vi "Write CE BT Hop Number Setting.vi"(8 "error in (no error)":errorcluster, 10 "CE BT Hop Number Setting":T1 {"Start/Stop Frequency(Hz)"."Stop" format="%#_6p"; "Start/Stop Frequency(Hz)"."Start" format="%#_6p"; "Sweep Time(s)"."Time" format="%#_6p"; "RBW/VBW(Hz)"."VBW" format="%#_6p"; "RBW/VBW(Hz)"."RBW" format="%#_6p"}, 11 "SA Measurement in":refnum<class "SA Measurement.lvclass">) -> (0 "error out":errorcluster, 3 "SA Measurement out":refnum<class "SA Measurement.lvclass">)   [LabVIEW 2023, in "Spectrum Analyzer.lvlib" / "SA Measurement.lvclass"]
uses:
  SA Measurement.lvclass
  SA Measurement.lvclass/SA Measurement.ctl
  TYPE DEFINITION/TYPE Reference Level and Atten Param.ctl
  Spectrum Analyzer.lvlib
  TYPE DEFINITION/TYPE Y-axis Unit.ctl
  TYPE DEFINITION/TYPE Display Trace Mode Select.ctl
  TYPE DEFINITION/TYPE Detect Mode Select.ctl
  TYPE DEFINITION/TYPE Average Mode Select.ctl
  TYPE DEFINITION/TYPE Start and Stop Frequency.ctl
  TYPE DEFINITION/SA Measurement Class/TYPE CE BT Hop Number Setting Param.ctl
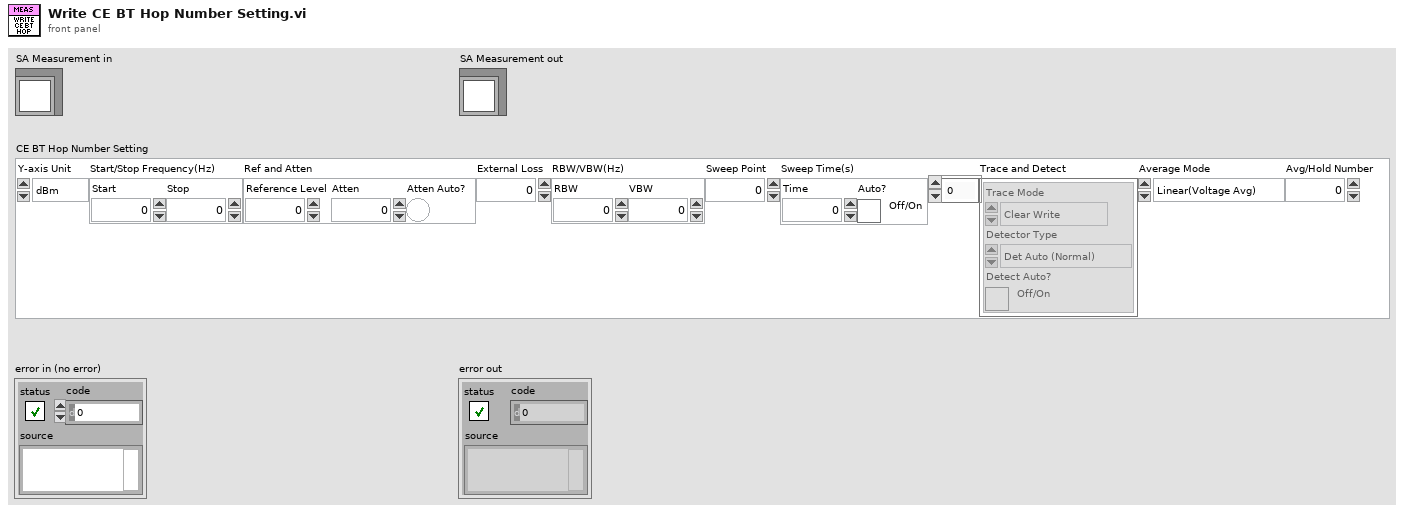
[diagram p1: front panel]
types:
  T1 = typedef "Spectrum Analyzer.lvlib/TYPE CE BT Hop Number Setting Param.ctl" = cluster{"Y-axis Unit":T2, "Start/Stop Frequency(Hz)":T3, "Ref and Atten":T4, "External Loss":dbl, "RBW/VBW(Hz)":cluster{"RBW":dbl, "VBW":dbl}, "Sweep Point":u32, "Sweep Time(s)":cluster{"Time":dbl, "Auto?":bool}, "Trace and Detect":cluster{"Trace Mode":T5, "Detector Type":T6, "Detect Auto?":bool}[], "Average Mode":T7, "Avg/Hold Number":u32}
  T2 = typedef "Spectrum Analyzer.lvlib/TYPE Y-axis Unit.ctl" = enum16{"dBm", "dBmV", "dBuV", "dBpW", "Volt", "Ampere", "Watt"}
  T3 = typedef "Spectrum Analyzer.lvlib/TYPE Start and Stop Frequency.ctl" = cluster{"Start":dbl, "Stop":dbl}
  T4 = typedef "Spectrum Analyzer.lvlib/TYPE Reference Level and Atten Param.ctl" = cluster{"Reference Level":dbl, "Atten":i32, "Atten Auto?":bool}
  T5 = typedef "Spectrum Analyzer.lvlib/TYPE Display Trace Mode Select.ctl" = enum16{"Clear Write", "Max Hold", "Min Hold", "Average", "View"}
  T6 = typedef "Spectrum Analyzer.lvlib/TYPE Detect Mode Select.ctl" = enum16{"Det Auto (Normal)", "Auto Peak", "Positive Peak", "Negative Peak", "Sample", "RMS", "Average", "Quasipeak", "CISPR Average", "RMS Average"}
  T7 = typedef "Spectrum Analyzer.lvlib/TYPE Average Mode Select.ctl" = enum16{"Linear(Voltage Avg)", "Video(Log)", "Power"}
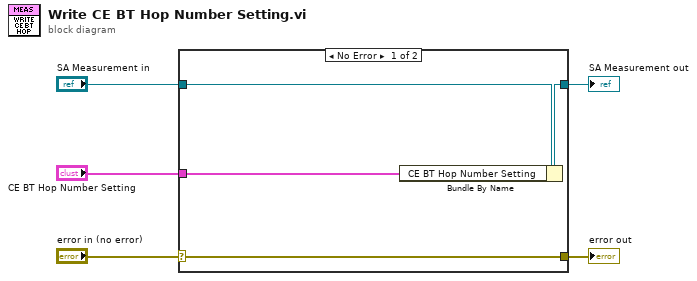
[diagram p0: block diagram]
diagram:
  n1 = case shown="No Error" "error in (no error)" {
    selector: "error in (no error)" -> [w9 w10]
    tunnel: [w9 w10] -> w4
    tunnel: [w7 w11] -> w2
    tunnel: "SA Measurement in" -> [w8 w11]
    tunnel: "CE BT Hop Number Setting" -> [w6 _]
    frame No Error {
      n2 = Bundle By Name(cluster=w8, "CE BT Hop Number Setting"=w6) -> (w7:refnum<class "SA Measurement.lvclass">)
    }
    frame Error {
    }
  }
  "error out" <- w4
  "SA Measurement out" <- w2
